vi "Host - Revert.vi"(8 "error in":errorcluster, 10 "Target IP Address in":string, 11 "Slave Ref in":refnum<k21>) -> (0 "error out":errorcluster, 1 "Message output":string, 2 "Target IP Address out":string, 3 "Slave Ref out":refnum<k21>)   [LabVIEW 2020, in "SEECD System Explorer.lvlib"]
uses:
  SEECD System Explorer.lvlib
  <vilib>/Utility/sysdir.llb/Get System Directory.vi
  <resource>/objmgr/IndComECAT.rc
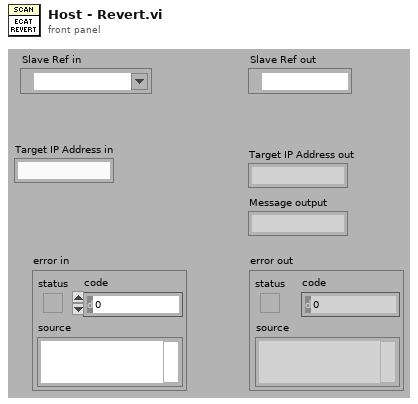
[diagram p1: front panel]
types:
  T1 = enum16{"open", "replace", "create", "open or create", "replace or create", "replace or create with confirmation"}
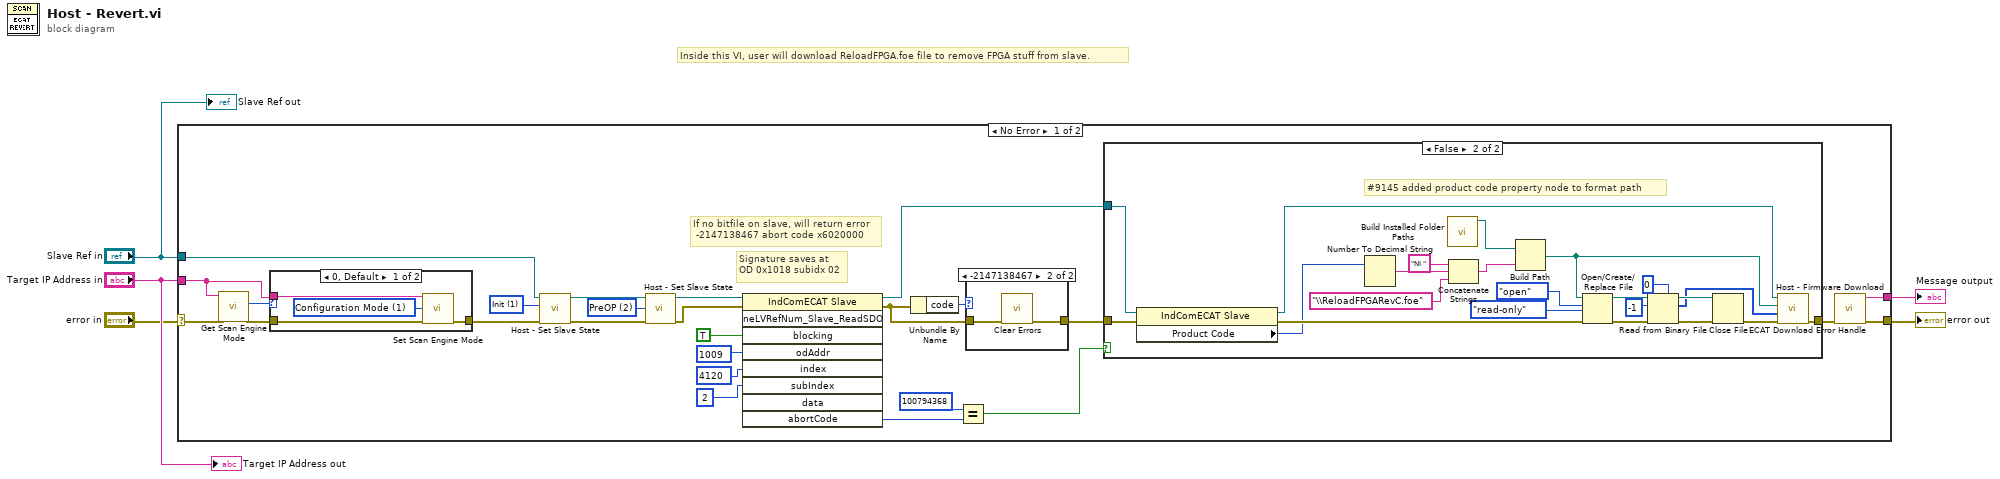
[diagram p0: block diagram]
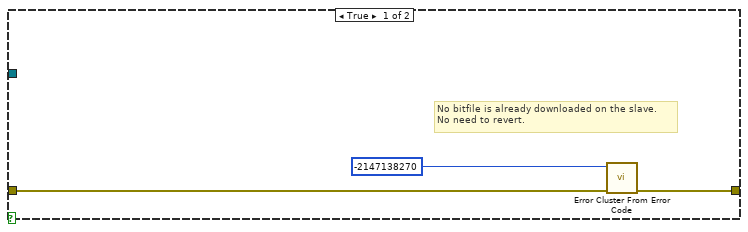
[diagram p3: hidden frame]
diagram:
  # "Inside this VI, user will download ReloadFPGA.foe file to remove FPGA stuff from slave."
  n1 = case shown="No Error" "error in" {
    selector: "error in" -> [w26 w65]
    tunnel: [w30 w65] -> w5
    tunnel: "Target IP Address in" -> [w25 _]
    tunnel: "Slave Ref in" -> [w29 _]
    tunnel: [w6 _] -> w1
    frame No Error {
      w21 = u32 2 items=["Init"=1, "PreOP"=2, "BootStrap"=3, "SafeOP"=4, "OP"=8] ("slaveState")
      w20 = u32 1 items=["Init"=1, "PreOP"=2, "BootStrap"=3, "SafeOP"=4, "OP"=8] ("slaveState")
      # "If no bitfile on slave, will return error\n -2147138467 abort code x6020000"
      # "Signature saves at \nOD 0x1018 subidx 02"
      n2 = call <vilib>:"Get Scan Engine Mode.vi"("error in (no error)"=w26, "target address (localhost)"=w25) -> ("error out"=w27:errorcluster, "mode"=w28:i32)  [unwired: 8 in]
      n3 = case shown="0, Default" w28 {
        tunnel: w25 -> [w62 _]
        tunnel: w27 -> [w61 w64]
        tunnel: [w60 w64] -> w24
        frame 0, Default {
          w63 = 1 items=["Configuration Mode"=1, "Active Mode"=2] ("mode (Active Mode)")
          n4 = call <vilib>:"Set Scan Engine Mode.vi"("target address (localhost)"=w62, "mode (Active Mode)"=w63, "error in (no error)"=w61) -> ("error out"=w60:errorcluster)  [unwired: 12 in]
        }
        frame 1 {
        }
      }
      n5 = call "Host - Set Slave State.vi"("error in (no error)"=w24, "slaveState"=w20, "Slave Ref in"=w29) -> ("error out"=w23:errorcluster, "Slave Ref out"=w22:refnum<k21>)  [unwired: 5 in, 2 out]
      n6 = call "Host - Set Slave State.vi"("error in (no error)"=w23, "slaveState"=w21, "Slave Ref in"=w22) -> ("error out"=w18:errorcluster, "Slave Ref out"=w19:refnum<k21>)  [unwired: 5 in, 2 out]
      n7 = invoke class="IndComECAT Slave" method="neLVRefNum_Slave_ReadSDO"(reference=w19, error in=w18, "blocking"=TRUE, "odAddr"=u16 1009, "index"=u16 4120, "subIndex"=u8 2) -> (reference out=w15:refnum<k21>, error out=w9:errorcluster, "abortCode"=w8:u32)  [unwired: 3 in, 6 out]
      n8 = Unbundle By Name(w9) -> ("code"=w10:i32)
      n9 = Equal?(x=u32 100794368 ("Numeric 2"), y=w8) -> (x = y?=w17:bool)
      n10 = case shown="-2147138467" w10 {
        tunnel: w9 -> [w32 w34]
        tunnel: [w32 w33] -> w16
        frame 0, Default {
        }
        frame -2147138467 {
          n11 = call <vilib>:"Clear Errors.vi"("error in (no error)"=w34) -> ("error out"=w33:errorcluster)  [unwired: 5 in, 1 out]
        }
      }
      n12 = case shown="False" w17 {
        tunnel: [w35 w47] -> w31
        tunnel: w16 -> [w36 w59]
        tunnel: w15 -> [_ w45]
        frame True {
          # "No bitfile is already downloaded on the slave.\nNo need to revert."
          n13 = call <vilib>:"Error Cluster From Error Code.vi"("error in (no error)"=w36, "error code (0)"=-2147138270) -> ("error out"=w35:errorcluster)  [unwired: 7 in]
        }
        frame False {
          # "#9145 added product code property node to format path"
          n14 = property class="IndComECAT Slave"(reference=w45, error in=w59) -> (reference out=w39:refnum<k21>, error out=w46:errorcluster, "Product Code"=w40:u32)
          n15 = Number To Decimal String(number=w40) -> (decimal integer string=w44:string)  [unwired: 1 in]
          n16 = call "Build Installed Folder Paths.vi"() -> ("Data Folder Path"=w38:path)  [unwired: 10 in, 1 out]
          n17 = Concatenate Strings("NI " ("string"), w44, "\\ReloadFPGARevC.foe" ("name or relative path")) -> (w41:string)
          n18 = Build Path(base path=w38, name or relative path=w41) -> (appended path=w49:path)
          n19 = Open/Create/Replace File(file path (use dialog)=w49, error in=w46, operation (0:open)=T1."open", access (0:read/write)=enum16{"read/write", "read-only", "write-only"}."read-only") -> (refnum out=w55:refnum<file>, error out=w56:errorcluster)  [unwired: 2 in, 1 out]
          n20 = Read from Binary File(5:u8 0, 8:w56, 10:-1 ("count (1)"), 11:w55) -> (0:w53:errorcluster, 2:w50:u8[], 3:w52:refnum<file>)  [unwired: 2 in, 1 out]
          n21 = Close File(refnum=w52, error in=w53) -> (error out=w48:errorcluster)  [unwired: 1 out]
          n22 = call "Host - Firmware Download.vi"("error in (no error)"=w48, "File Byte Array"=w50, "Firmware filename"=w49, "Slave Ref in"=w39) -> ("error out"=w47:errorcluster)  [unwired: 7 in]
        }
      }
      n23 = call "ECAT Download Error Handle.vi"("error in"=w31) -> ("error out"=w30:errorcluster, "Message output"=w6:string)  [unwired: 9 in]
    }
    frame Error {
    }
  }
  "error out" <- w5
  "Message output" <- w1
  "Target IP Address out" <- "Target IP Address in"
  "Slave Ref out" <- "Slave Ref in"
